vi "Test_Stop_Midrun.vi"(8 "error in":errorcluster, 11 "Sequence Path":path=path "C:/Users/DynaAdmin/PycharmProjects/Universal-sequence-executor-AF/configs/sequences/vtu_actual_sequence.json") -> (0 "error out":errorcluster)   [LabVIEW 2026]
doc: "Stop test: Load -> Start -> wait 3s (mid-run) -> Send Stop Sequence -> wait 2s -> Normal Stop -> notify. Evidence: results/trace_abort.txt = AB|STOPPED BY OPERATOR."
uses:
  src/Executor/Sequence Executor.lvclass
  src/Executor Messages/Load Sequence Msg/Load Sequence Msg.lvclass/Load Sequence Msg.ctl
  <vilib>/ActorFramework/Message Enqueuer/Message Enqueuer.lvclass/Message Enqueuer.ctl
  <vilib>/ActorFramework/Message Enqueuer/Enqueue.vi
  src/Executor Messages/Load Sequence Msg/Load Sequence Msg.lvclass
  src/Executor Messages/Start Sequence Msg/Start Sequence Msg.lvclass
  src/Executor Messages/Stop Sequence Msg/Stop Sequence Msg.lvclass
  <vilib>/ActorFramework/Stop Msg/Stop Msg.lvclass
  <vilib>/ActorFramework/Message Priority Queue/Priority Enqueue.vi
  <vilib>/ActorFramework/Actor/Actor.lvclass
panel:
  out "Stop Seq error":errorcluster
  out "Stopped cleanly":bool
  out "Feedback Chart":dbl
  out "Verdict":string
  out "Channel Values":string[][](array[string])
  out "Step Table":string[][](array[string])
  out "Step Index":i32
  out "Status":string
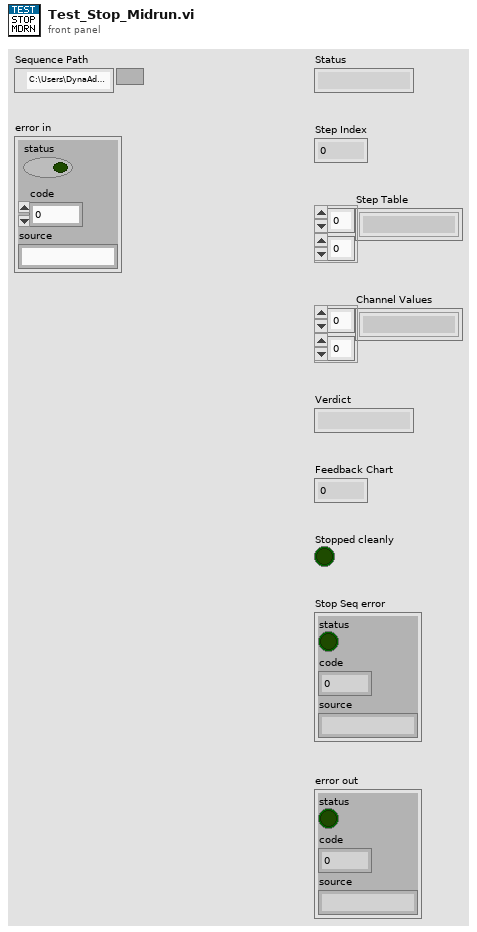
[diagram p1: front panel]
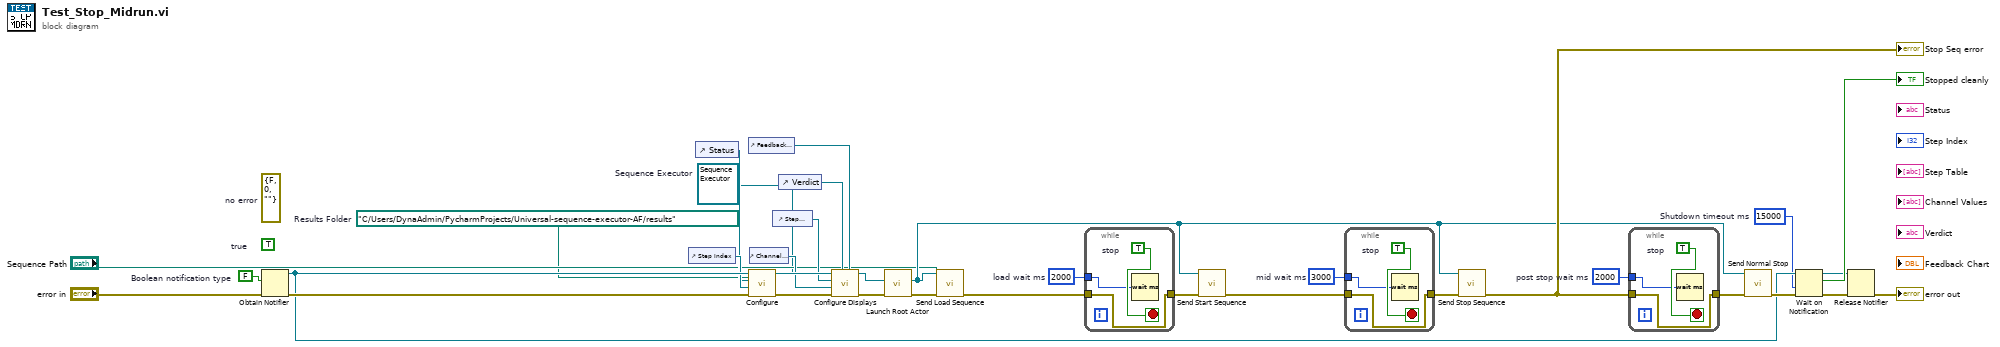
[diagram p0: block diagram]
diagram:
  w7 = 2000  # post stop wait ms
  w6 = 3000  # mid wait ms
  w5 = 2000  # load wait ms
  (unwired) TRUE  # true
  w4 = path "C:/Users/DynaAdmin/PycharmProjects/Universal-sequence-executor-AF/results"  # Results Folder
  w3 = 15000  # Shutdown timeout ms
  (unwired) errorcluster {"status"=FALSE, "code"=0, "source"=""}  # no error
  w2 = FALSE  # Boolean notification type
  w1 = refnum<class "Sequence Executor.lvclass"> refnum  # Sequence Executor
  n1 = Obtain Notifier(notification data type=w2, error in (no error)="error in") -> (notifier out=w16:refnum<notifier>, error out=w17:errorcluster)  [unwired: 2 in, 1 out]
  n2 = control-ref of="Step Index"() -> (w11:refnum<vi>)
  n3 = control-ref of="Status"() -> (w10:refnum<vi>)
  n4 = control-ref of="Feedback Chart"() -> (w15:refnum<vi>)
  n5 = call "Configure.vi"("Results Folder"=w4, "Stopped Notification"=w16, "error in"=w17, "Step Index Display"=w11, "Status Display"=w10, "Sequence Executor in"=w1) -> ("error out"=w19:errorcluster, "Sequence Executor out"=w18:refnum<class "Sequence Executor.lvclass">)  [unwired: 4 in]
  n6 = control-ref of="Channel Values"() -> (w13:refnum<vi>)
  n7 = control-ref of="Step Table"() -> (w12:refnum<vi>)
  n8 = control-ref of="Verdict"() -> (w14:refnum<vi>)
  n9 = call "Configure Displays.vi"("Feedback Chart"=w15, "Verdict Display"=w14, "error in"=w19, "Channel Values Display"=w13, "Step Table Display"=w12, "Sequence Executor in"=w18) -> ("error out"=w21:errorcluster, "Sequence Executor out"=w20:refnum<class "Sequence Executor.lvclass">)  [unwired: 4 in]
  n10 = call <vilib>:"Launch Root Actor.vi"("error in (no error)"=w21, "Actor"=w20) -> ("error out"=w23:errorcluster, "Actor's Enqueuer"=w22:refnum<class "Message Enqueuer.lvclass">)  [unwired: 8 in]
  n11 = call "Send Load Sequence.vi"("error in (no error)"=w23, "path"="Sequence Path", "Message Enqueuer"=w22) -> ("error out"=w24:errorcluster)  [unwired: 7 in, 1 out]
  n12 = while {
    tunnel: w5 -> [w36]
    tunnel: w24 -> [w35]
    tunnel: [w35] -> w25
    stop <- w37 stop-if-true
    w37 = TRUE  # stop
    n13 = Wait (ms)(milliseconds to wait=w36) -> ()  [unwired: 1 out]
  }
  n14 = call "Send Start Sequence.vi"("error in (no error)"=w25, "Message Enqueuer"=w22) -> ("error out"=w26:errorcluster)  [unwired: 8 in, 1 out]
  n15 = while {
    tunnel: w6 -> [w39]
    tunnel: w26 -> [w38]
    tunnel: [w38] -> w27
    stop <- w40 stop-if-true
    w40 = TRUE  # stop
    n16 = Wait (ms)(milliseconds to wait=w39) -> ()  [unwired: 1 out]
  }
  n17 = call "Send Stop Sequence.vi"("error in (no error)"=w27, "Message Enqueuer"=w22) -> ("error out"=w28:errorcluster)  [unwired: 8 in, 1 out]
  "Stop Seq error" <- w28
  n18 = while {
    tunnel: w7 -> [w42]
    tunnel: w28 -> [w41]
    tunnel: [w41] -> w29
    stop <- w43 stop-if-true
    w43 = TRUE  # stop
    n19 = Wait (ms)(milliseconds to wait=w42) -> ()  [unwired: 1 out]
  }
  n20 = call <vilib>:"Send Normal Stop.vi"("error in (no error)"=w29, "Message Enqueuer"=w22) -> ("error out"=w30:errorcluster)  [unwired: 9 in]
  n21 = Wait on Notification(notifier=w16, timeout in ms (-1)=w3, error in (no error)=w30) -> (notifier out=w31:refnum<notifier>, notification=→"Stopped cleanly":bool, error out=w33:errorcluster)  [unwired: 1 in, 1 out]
  n22 = Release Notifier(notifier=w31, error in (no error)=w33) -> (error out=→"error out":errorcluster)  [unwired: 1 in, 2 out]
